vi "ResampleXY.vi"(6 "Interpolation Method":i32(ring)=2 items=["nearest", "linear", "spline", "cubic Hermite", "Lagrange"], 7 "Interpolation Distance":dbl format="%#_13g", 8 "error in (no error)":errorcluster, 9 "t":dbl[](array[numeric]), 10 "Y":dbl[](array[numeric]), 11 "X":dbl[](array[numeric])) -> (0 "error out":errorcluster, 2 "Resampled Y":dbl[](array[numeric]), 3 "Resampled X":dbl[](array[numeric]))   [LabVIEW 2019, in "Tool Object.lvclass"]
uses:
  Tool Object.lvclass
  <vilib>/Analysis/1siggen.llb/Ramp Pattern by Samples.vi
  <vilib>/gmath/NI_Gmath.lvlib
  <vilib>/Analysis/NI_AALBase.lvlib
  Tool Path/Tool Path.lvclass
panel:
  out "XY Graph":cluster{"X":dbl[], "Y":dbl[]}(graph)
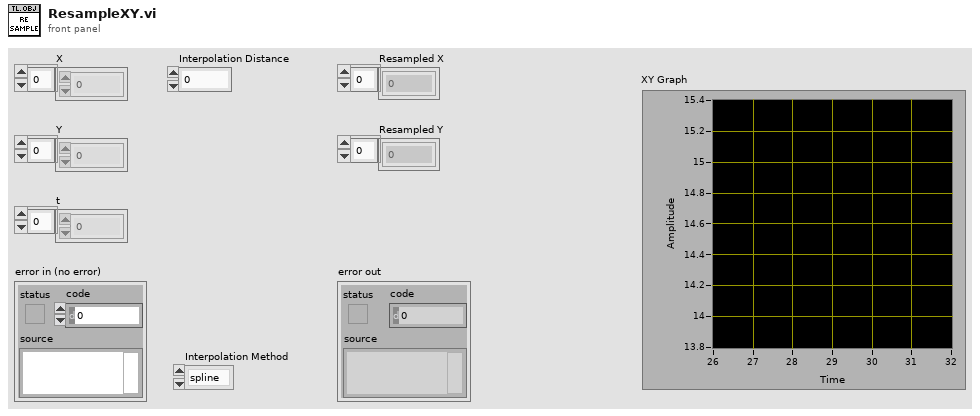
[diagram p1: front panel]
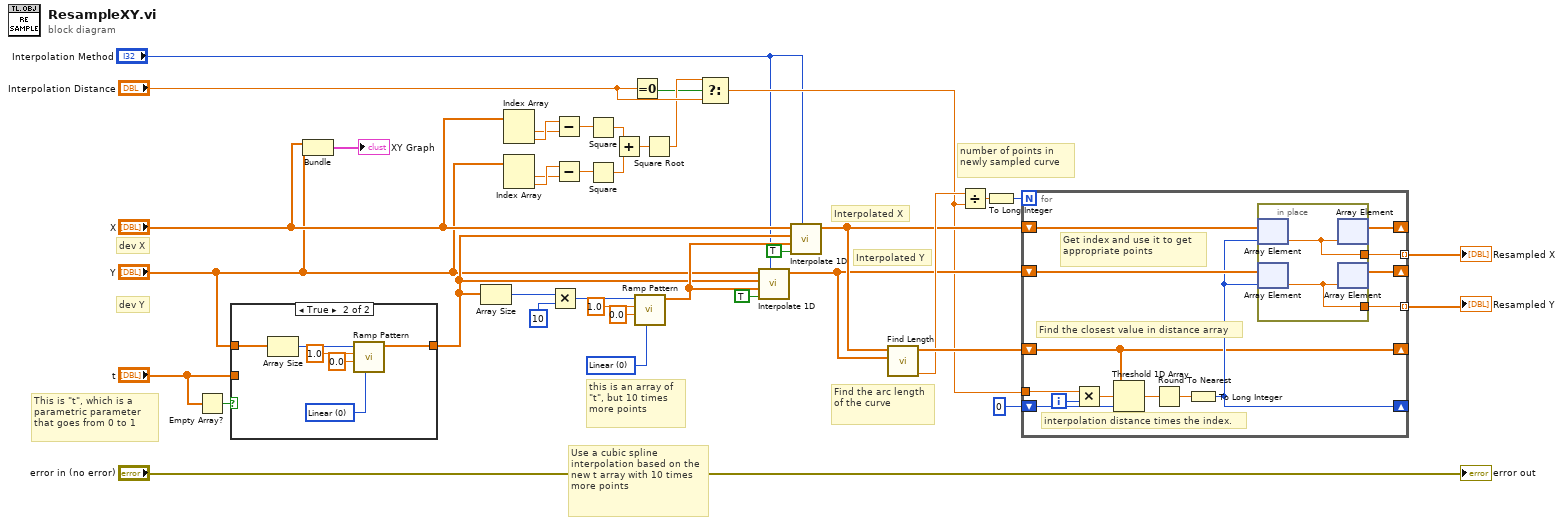
[diagram p0: block diagram]
diagram:
  w37 = u16 0 items=["Linear", "Logarithmic"] ("type")
  # "number of points in newly sampled curve"
  # "Find the arc length of the curve"
  # "Use a cubic spline interpolation based on the new t array with 10 times more points"
  # "this is an array of \"t\", but 10 times more points"
  # "dev X"
  # "dev Y"
  # "This is \"t\", which is a parametric parameter that goes from 0 to 1"
  # "Interpolated Y"
  # "Interpolated X"
  n1 = Empty Array?(array="t") -> (empty?=w21:bool)
  n2 = case shown="True" w21 {
    tunnel: "t" -> [w40 _]
    tunnel: [w40 w42] -> w14
    tunnel: "Y" -> [_ w41]
    frame False {
    }
    frame True {
      w46 = u16 0 items=["Linear", "Logarithmic"] ("type")
      n3 = Array Size(array=w41) -> (size(s)=w43:i32)
      n4 = call-poly <vilib>:"Ramp Pattern.vi"("type"=w46, "start"=0.0, "end"=1.0, "samples"=w43) -> ("Ramp Pattern"=w42:dbl[])  [unwired: 6 in, 1 out]
    }
  }
  n5 = Bundle("X"="X", "Y"="Y") -> (→"XY Graph":cluster{"X":dbl[], "Y":dbl[]})  [unwired: 1 in]
  n6 = Array Size(array=w14) -> (size(s)=w27:i32)
  n7 = Index Array(array="X") -> (element #1=w12:dbl, element #2=w13:dbl)  [unwired: 2 in]
  n8 = Index Array(array="Y") -> (element #1=w10:dbl, element #2=w11:dbl)  [unwired: 2 in]
  n9 = Multiply(x=w27, y=10 ("x")) -> (x*y=w33:i32)
  n10 = Subtract(x=w13, y=w12) -> (x-y=w8:dbl)
  n11 = Subtract(x=w11, y=w10) -> (x-y=w9:dbl)
  n12 = Square(x=w8) -> (x^2=w7:dbl)
  n13 = Square(x=w9) -> (x^2=w6:dbl)
  n14 = Add(x=w7, y=w6) -> (x+y=w5:dbl)
  n15 = Equal To 0?(x="Interpolation Distance") -> (x = 0?=w3:bool)
  n16 = call-poly <vilib>:"Ramp Pattern.vi"("type"=w37, "start"=0.0, "end"=1.0, "samples"=w33) -> ("Ramp Pattern"=w32:dbl[])  [unwired: 6 in, 1 out]
  n17 = Square Root(x=w5) -> (sqrt(x)=w4:dbl)
  n18 = Select(t=w4, s=w3, f="Interpolation Distance") -> (s? t:f=w16:dbl)
  n19 = call <vilib>:"Interpolate 1D.vi"("method"="Interpolation Method", "X is monotonic"=TRUE, "xi"=w32, "X"=w14, "Y"="Y") -> ("yi"=w30:dbl[])  [unwired: 4 in, 2 out]
  n20 = call <vilib>:"Interpolate 1D.vi"("method"="Interpolation Method", "X is monotonic"=TRUE, "xi"=w32, "X"=w14, "Y"="X") -> ("yi"=w31:dbl[])  [unwired: 4 in, 2 out]
  n21 = call "Find Length.vi"("Y"=w30, "X"=w31) -> ("Total Length"=w34:dbl, "Cumulative Length"=w35:dbl[])  [unwired: 6 in, 2 out]
  n22 = Divide(x=w34, y=w16) -> (x/y=w25:dbl)
  n23 = To Long Integer(number=w25) -> (32bit integer=w24:i32)
  n24 = for {
    N: w24 -> [_]
    tunnel: w16 -> [w60]
    shift-right: [w55] -> _
    shift-left: w31 -> [w57]
    shift-right: [w54] -> _
    shift-left: w30 -> [w56]
    tunnel: [w53] -> w22 mode=indexing
    tunnel: [w52] -> w23 mode=indexing
    shift-right: [w47] -> _
    shift-left: w35 -> [w47]
    shift-right: [w50] -> _
    shift-left: 0 -> [w51]
    i -> [w59]
    # "interpolation distance times the index."
    # "Get index and use it to get appropriate points"
    # "Find the closest value in distance array"
    n25 = Multiply(x=w60, y=w59) -> (x*y=w58:dbl)
    n26 = Threshold 1D Array(1:w51, 2:w58, 3:w47) -> (0:w49:dbl)
    n27 = Round To Nearest(number=w49) -> (nearest integer value=w48:dbl)
    n28 = To Long Integer(number=w48) -> (32bit integer=w50:i32)
    n29 = in-place {
      in-place-border: [w62] -> w52
      in-place-border: [w61] -> w53
      n30 = in-place-array #1(w57, w50) -> (w62:dbl)
      n31 = in-place-array #2(w56, w50) -> (w61:dbl)
      n32 = in-place-array #1(w62) -> (w55:dbl[])  [unwired: 1 out]
      n33 = in-place-array #2(w61) -> (w54:dbl[])  [unwired: 1 out]
    }
  }
  "Resampled Y" <- w22
  "Resampled X" <- w23
  "error out" <- "error in (no error)"
